vi "AT1B_Ultraschall.vi"() -> ()   [LabVIEW 2026]
doc: "Virtueller Sensor. Teach-Taste einschalten = halten, ausschalten = loslassen. Messgeraeteskala bleibt fest. Bewegung, Messung und Aufnahme sind getrennt schaltbar.\nModellgrenzen stehen in der Anleitung."
panel:
  out "Bewegungsparameter gueltig":bool=TRUE
  out "Grafikfehlercode":i32
  out "Stromverlauf [mA] - 20 ms je Punkt":dbl(graph)
  out "CSV-Fehlercode":i32
  out "Ungespeicherte Daten":bool
  out "Zeilen aufgenommen":i32
  out "Aufnahmestatus":string
  in  "Pruefstand beenden":bool
  in  "Neue CSV-Datei":path
  in  "CSV speichern":bool
  in  "Ungespeicherte Aufnahme verwerfen erlauben":bool
  in  "Neue Aufnahme":bool
  in  "Aufnahme eingeschaltet":bool
  out "Schaltausgang invertiert":bool
  out "Signalzustand":string="Mit Ausfuehren / Strg+R starten."
  out "Messung angehalten - Anzeige historisch":bool
  out "Status-LED":bool
  out "Status-LED [Hz]":dbl=nan
  out "Taste gehalten [s]":dbl=nan
  out "Teach-Phase [0 / 1 / 2]":dbl=nan
  out "Echo-LED":bool
  out "OUT1 - orange":bool
  out "Messgeraet [mm] - feste Skala":dbl=nan
  out "Strom [mA]":dbl=nan
  in  "Messung eingeschaltet":bool=TRUE
  in  "Rausch-Startwert [1..2147483646]":dbl=1.0
  in  "Schalthysterese [mm] - Beispiel":dbl=3.0
  in  "Rauschamplitude [mm] - Beispiel":dbl
  in  "Messoffset [mm] - Beispiel":dbl
  in  "Teach-Taste gedrueckt":bool
  in  "Echo vorhanden":bool=TRUE
  in  "Sensor eingeschaltet":bool=TRUE
  out "Abgeschlossene Fahrten":dbl
  out "Fahrt aktiv":bool
  out "Position aktuell":dbl
  in  "Bewegung pausieren":bool
  in  "Bewegung stoppen":bool
  in  "Ablauf starten":bool
  in  "Schrittweite":dbl=1.0
  in  "Fahrtart":enum16{"Pendeln", "Schritte", "Einfachfahrt"}(ring)
  in  "Wiederholungen":dbl=1.0
  in  "Haltezeit [s]":dbl=0.5
  in  "Tempo pro Sekunde":dbl=25.0
  in  "Endposition":dbl=400.0
  in  "Startposition":dbl=50.0
  in  "Position setzen":bool
  in  "Handposition":dbl=250.0
  out "Kurzhilfe":string="Virtueller Sensor. Teach-Taste einschalten = halten, ausschalten = loslassen. Messgeraeteskala bleibt fest. Bewegung, Messung und Aufnahme sind getrennt schaltbar.\nModellgrenzen stehen in der Anleitung."
  out "Pruefstand":string="AT-1B / Ultraschall AU004 - Wegwerte in mm"
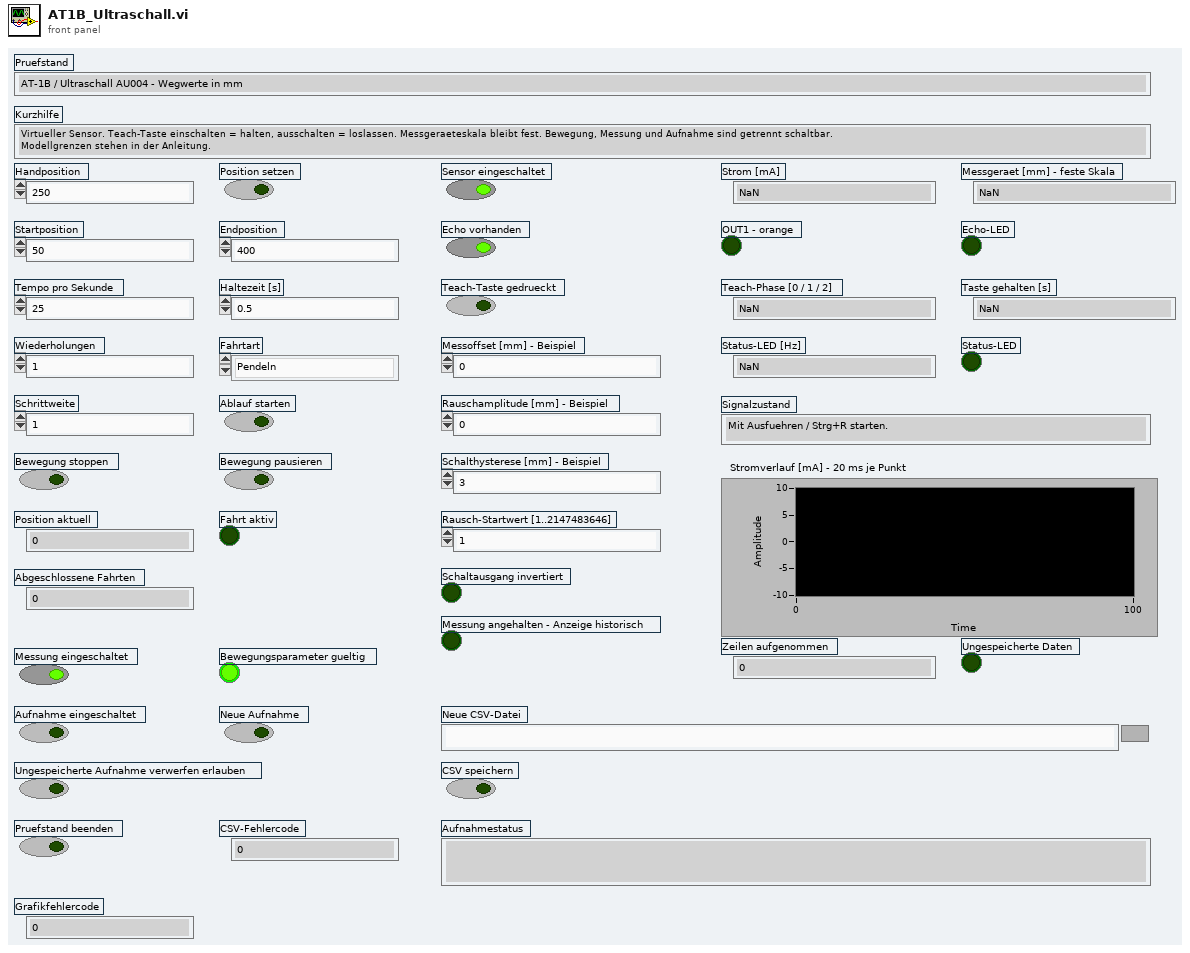
[diagram p1: front panel]
types:
  T1 = cluster{"record":bool, "clear":bool, "limit":i32, "header":string, "source":string}
diagram:
  n1 = while {
    shift-right: [w27] -> _
    shift-left: dbl[] [0.0, 0.0, 0.0, 0.0, 0.0, 0.0, 0.0, 0.0, 0.0, 0.0, 0.0, 0.0] -> [w26]
    shift-right: [w75] -> _
    shift-left: dbl[] [0.0, 0.0, 0.0, 0.0, 0.0, 0.0, 0.0, 0.0, 0.0, 0.0, 0.0, 0.0, 0.0, 0.0, 0.0, 0.0] -> [w74]
    shift-right: [w80] -> _
    shift-left: dbl[] [nan, nan, nan, nan, nan, nan, nan, nan] -> [w79]
    shift-right: [w162] -> _
    shift-left: cluster{"text":string, "count":i32} {"text"="Quelle;Zeit_s;Position_mm;Strom_mA;Anzeige_mm;OUT1;EchoLED;Qualitaet;Teachphase;Taste_s;LED_Hz;Invertiert;StatusLED;Eingang_dt_s;Eingang_distance_mm;Eingang_echo_present;Eingang_power;Eingang_teach_pressed;Eingang_offset_mm;Eingang_noise_amplitude_mm;Eingang_resolution_mm;Eingang_hysteresis_mm_example;Eingang_teach_timeout_s_example;Eingang_noise_seed\r\n", "count"=0} -> [w161]
    shift-right: [w164] -> _
    shift-left: 0 -> [w163]
    shift-right: [w207] -> _
    shift-left: errorcluster {"status"=FALSE, "code"=0, "source"=""} -> [w206]
    i -> [w7]
    stop <- w223 stop-if-true
    w10 = FALSE
    (unwired) 1.0
    w9 = 0.0
    w8 = 0.02
    # "Virtueller Pruefstand - 20 ms Modellschritt"
    n2 = case shown="True" "Position setzen" {
      frame False {
      }
      frame True {
        n3 = property on="Position setzen" class="Bool. (strikt)"("Value"=FALSE) -> ()  [unwired: 2 in, 2 out]
      }
    }
    n4 = case shown="True" "Ablauf starten" {
      frame False {
      }
      frame True {
        n5 = property on="Ablauf starten" class="Bool. (strikt)"("Value"=FALSE) -> ()  [unwired: 2 in, 2 out]
      }
    }
    n6 = case shown="True" "Bewegung stoppen" {
      frame False {
      }
      frame True {
        n7 = property on="Bewegung stoppen" class="Bool. (strikt)"("Value"=FALSE) -> ()  [unwired: 2 in, 2 out]
      }
    }
    n8 = case shown="True" "Neue Aufnahme" {
      frame False {
      }
      frame True {
        n9 = property on="Neue Aufnahme" class="Bool. (strikt)"("Value"=FALSE) -> ()  [unwired: 2 in, 2 out]
      }
    }
    n10 = case shown="True" "CSV speichern" {
      frame False {
      }
      frame True {
        n11 = property on="CSV speichern" class="Bool. (strikt)"("Value"=FALSE) -> ()  [unwired: 2 in, 2 out]
      }
    }
    n12 = case shown="True" "Pruefstand beenden" {
      frame False {
      }
      frame True {
        n13 = property on="Pruefstand beenden" class="Bool. (strikt)"("Value"=FALSE) -> ()  [unwired: 2 in, 2 out]
      }
    }
    n14 = Wait (ms)(milliseconds to wait=u32 20) -> ()  [unwired: 1 out]
    n15 = Select(t=1.0, s="Ablauf starten", f=0.0) -> (s? t:f=w30:dbl)
    n16 = Select(t=1.0, s="Bewegung pausieren", f=0.0) -> (s? t:f=w33:dbl)
    n17 = Select(t=1.0, s="Position setzen", f=0.0) -> (s? t:f=w36:dbl)
    n18 = Select(t=1.0, s="Bewegung stoppen", f=0.0) -> (s? t:f=w39:dbl)
    n19 = Select(t=1.0, s="Echo vorhanden", f=0.0) -> (s? t:f=w65:dbl)
    n20 = property on="Stromverlauf [mA] - 20 ms je Punkt" class="SVDiagr (strikt)"("Legend:Visible"=w10, "Palette:Visible"=w10, "Scale Legend:Visible"=w10, "Position"=cluster{"Left":i32, "Top":i32} {"Left"=735, "Top"=420}, "Plot Area:Size"=cluster{"Width":u32, "Height":u32} {"Width"=340, "Height"=110}) -> (error out=w241:errorcluster)  [unwired: 2 in, 1 out]
    n21 = Select(t=1.0, s="Sensor eingeschaltet", f=0.0) -> (s? t:f=w68:dbl)
    n22 = Select(t=1.0, s="Teach-Taste gedrueckt", f=0.0) -> (s? t:f=w71:dbl)
    n23 = Not(x="Messung eingeschaltet") -> (.not. x?=→"Messung angehalten - Anzeige historisch":bool)
    n24 = And(x="Aufnahme eingeschaltet", y="Messung eingeschaltet") -> (x .and. y?=w173:bool)
    n25 = Unbundle By Name(w161) -> ("count"=w165:i32)  [unwired: 1 out]
    n26 = Equal?(x=w7, y=w9) -> ()  [unwired: 1 out]
    n27 = Quotient & Remainder(x=w7, y=5) -> (x-y*floor(x/y)=w171:i32)  [unwired: 1 out]
    n28 = Build Array(w8, "Startposition", "Endposition", "Tempo pro Sekunde", "Haltezeit [s]", "Wiederholungen", w30, w33, w36, "Handposition", "Fahrtart", "Schrittweite", w39) -> (w40:dbl[])
    n29 = Unbundle By Name(w241) -> ("code"=→"Grafikfehlercode":i32)
    n30 = Greater?(x=w165, y=w163) -> (0:w166:bool)
    n31 = Equal?(x=w171, y=w9) -> (x = y?=w172:bool)
    n32 = call "Trajektorie.vi"("StateIn"=w26, "Parameters"=w40) -> ("Values"=w41:dbl[], "StateOut"=w27:dbl[])  [unwired: 8 in]
    n33 = Not(x=w166) -> (.not. x?=w167:bool)
    n34 = And(x=w173, y=w172) -> (x .and. y?=w174:bool)
    n35 = Index Array(array=w41, index=0) -> (element=w43:dbl)
    "Position aktuell" <- w43
    n36 = Index Array(array=w41, index=3) -> (element=w45:dbl)
    n37 = Index Array(array=w41, index=4) -> (element=w47:dbl)
    n38 = Index Array(array=w41, index=1) -> (element=w51:dbl)
    n39 = Index Array(array=w41, index=2) -> (element=→"Abgeschlossene Fahrten":dbl)
    n40 = Or(x=w167, y="Ungespeicherte Aufnahme verwerfen erlauben") -> (x .or. y?=w168:bool)
    n41 = Greater?(x=w47, y=0.0) -> (0:→"Bewegungsparameter gueltig":bool)
    n42 = Greater?(x=w51, y=0.0) -> (0:→"Fahrt aktiv":bool)
    n43 = Build Array(w8, w43, w65, w68, w71, "Messoffset [mm] - Beispiel", "Rauschamplitude [mm] - Beispiel", 3.0, "Schalthysterese [mm] - Beispiel", 30.0, "Rausch-Startwert [1..2147483646]") -> (w76:dbl[])
    n44 = And(x="Neue Aufnahme", y=w168) -> (x .and. y?=w169:bool)
    n45 = Not(x=w168) -> (.not. x?=w224:bool)
    n46 = call "AU004_Schritt.vi"("StateIn"=w74, "Parameters"=w76) -> ("Values"=w77:dbl[], "StateOut"=w75:dbl[])  [unwired: 8 in]
    n47 = Index Array(array=w76, index=0) -> (element=w181:dbl)
    n48 = Index Array(array=w76, index=1) -> (element=w183:dbl)
    n49 = Index Array(array=w76, index=2) -> (element=w185:dbl)
    n50 = Index Array(array=w76, index=3) -> (element=w187:dbl)
    n51 = Index Array(array=w76, index=4) -> (element=w189:dbl)
    n52 = Index Array(array=w76, index=5) -> (element=w191:dbl)
    n53 = Index Array(array=w76, index=6) -> (element=w193:dbl)
    n54 = Index Array(array=w76, index=7) -> (element=w195:dbl)
    n55 = Index Array(array=w76, index=8) -> (element=w197:dbl)
    n56 = Index Array(array=w76, index=9) -> (element=w199:dbl)
    n57 = Index Array(array=w76, index=10) -> (element=w201:dbl)
    n58 = Bundle By Name(cluster=T1 {"record"=FALSE, "clear"=FALSE, "limit"=10000, "header"="", "source"=""}, "record"=w174, "clear"=w169, "limit"=10000, "header"="Quelle;Zeit_s;Position_mm;Strom_mA;Anzeige_mm;OUT1;EchoLED;Qualitaet;Teachphase;Taste_s;LED_Hz;Invertiert;StatusLED;Eingang_dt_s;Eingang_distance_mm;Eingang_echo_present;Eingang_power;Eingang_teach_pressed;Eingang_offset_mm;Eingang_noise_amplitude_mm;Eingang_resolution_mm;Eingang_hysteresis_mm_example;Eingang_teach_timeout_s_example;Eingang_noise_seed\r\n", "source"="AT1B_Ultraschall;") -> (w179:T1)
    n59 = Select(t=errorcluster {"status"=FALSE, "code"=0, "source"=""}, s=w169, f=w206) -> (s? t:f=w212:errorcluster)
    n60 = Select(t=0, s=w169, f=w163) -> (s? t:f=w219:i32)
    n61 = And(x="Neue Aufnahme", y=w224) -> (x .and. y?=w225:bool)
    n62 = Select(t=w77, s="Messung eingeschaltet", f=w79) -> (s? t:f=w80:dbl[])
    n63 = Index Array(array=w77, index=3) -> (element=w86:dbl)
    n64 = Index Array(array=w77, index=4) -> (element=w90:dbl)
    n65 = Index Array(array=w77, index=14) -> (element=w100:dbl)
    n66 = Index Array(array=w77, index=5) -> (element=w105:dbl)
    n67 = Index Array(array=w77, index=12) -> (element=w132:dbl)
    n68 = Index Array(array=w77, index=0) -> (element=w136:dbl)
    n69 = Index Array(array=w77, index=1) -> (element=w138:dbl)
    n70 = Index Array(array=w77, index=3) -> (element=w140:dbl)
    n71 = Index Array(array=w77, index=4) -> (element=w142:dbl)
    n72 = Index Array(array=w77, index=5) -> (element=w144:dbl)
    n73 = Index Array(array=w77, index=6) -> (element=w146:dbl)
    n74 = Index Array(array=w77, index=7) -> (element=w148:dbl)
    n75 = Index Array(array=w77, index=8) -> (element=w150:dbl)
    n76 = Index Array(array=w77, index=12) -> (element=w152:dbl)
    n77 = Index Array(array=w77, index=14) -> (element=w154:dbl)
    n78 = Index Array(array=w80, index=0) -> (element=→"Strom [mA]":dbl)
    n79 = Index Array(array=w80, index=1) -> (element=→"Messgeraet [mm] - feste Skala":dbl)
    n80 = Greater?(x=w86, y=0.0) -> (0:→"OUT1 - orange":bool)
    n81 = Greater?(x=w90, y=0.0) -> (0:→"Echo-LED":bool)
    n82 = Index Array(array=w80, index=6) -> (element=→"Teach-Phase [0 / 1 / 2]":dbl)
    n83 = Index Array(array=w80, index=7) -> (element=→"Taste gehalten [s]":dbl)
    n84 = Index Array(array=w80, index=8) -> (element=→"Status-LED [Hz]":dbl)
    n85 = Greater?(x=w100, y=0.0) -> (0:→"Status-LED":bool)
    n86 = Equal?(x=w105, y=0.0) -> (x = y?=w108:bool)
    n87 = Equal?(x=w105, y=1.0) -> (x = y?=w112:bool)
    n88 = Equal?(x=w105, y=2.0) -> (x = y?=w116:bool)
    n89 = Equal?(x=w105, y=3.0) -> (x = y?=w120:bool)
    n90 = Equal?(x=w105, y=4.0) -> (x = y?=w124:bool)
    n91 = Equal?(x=w105, y=5.0) -> (x = y?=w128:bool)
    n92 = Greater?(x=w132, y=0.0) -> (0:→"Schaltausgang invertiert":bool)
    n93 = Build Array(w45, w43, w136, w138, w140, w142, w144, w146, w148, w150, w152, w154, w181, w183, w185, w187, w189, w191, w193, w195, w197, w199, w201) -> (w202:dbl[])
    n94 = Index Array(array=w80, index=0) -> (element=→"Stromverlauf [mA] - 20 ms je Punkt":dbl)
    n95 = Select(t="Messsignal gueltig", s=w108, f="Parameter ungueltig - Eingaben pruefen.") -> (s? t:f=w110:string)
    n96 = call "Aufzeichnung_Schritt.vi"("Previous"=w161, "Row"=w202, "Settings"=w179) -> ("Full"=w203:bool, "Current"=w162:cluster{"text":string, "count":i32})  [unwired: 11 in]
    n97 = Select(t="Noch keine Teachpunkte gespeichert", s=w112, f=w110) -> (s? t:f=w114:string)
    n98 = Unbundle By Name(w162) -> ("text"=w204:string, "count"=w205:i32)
    "Zeilen aufgenommen" <- w205
    n99 = Select(t="Abstand ausserhalb 50..400 mm", s=w116, f=w114) -> (s? t:f=w118:string)
    n100 = Greater?(x=w205, y=0.0) -> (0:w209:bool)
    n101 = Select(t="Kein Echo", s=w120, f=w118) -> (s? t:f=w122:string)
    n102 = And(x="CSV speichern", y=w209) -> (x .and. y?=w210:bool)
    n103 = case shown="True" w210 {
      tunnel: "Neue CSV-Datei" -> [_ w244]
      tunnel: w212 -> [w243 _]
      tunnel: w204 -> [_ w245]
      tunnel: [w243 w246] -> w207
      frame False {
      }
      frame True {
        n104 = call "CSV_Speichern.vi"("Text"=w245, "Datei"=w244) -> ("error out"=w246:errorcluster)  [unwired: 13 in]
      }
    }
    n105 = Select(t="Sensor laeuft an", s=w124, f=w122) -> (s? t:f=w126:string)
    n106 = Select(t="Sensor ausgeschaltet", s=w128, f=w126) -> (s? t:f=→"Signalzustand":string)
    n107 = Unbundle By Name(w207) -> ("status"=w213:bool, "code"=→"CSV-Fehlercode":i32, "source"=w215:string)
    n108 = Not(x=w213) -> (.not. x?=w216:bool)
    n109 = And(x=w210, y=w216) -> (x .and. y?=w217:bool)
    n110 = Select(t=w205, s=w217, f=w219) -> (s? t:f=w164:i32)
    n111 = Greater?(x=w205, y=w164) -> (0:w220:bool)
    "Ungespeicherte Daten" <- w220
    n112 = Not(x=w220) -> (.not. x?=w221:bool)
    n113 = Select(t="Aufnahme noch nicht gespeichert. Vor neuer Aufnahme oder Beenden CSV speichern oder Verwerfen erlauben einschalten.", s=w220, f="Bereit. Aufnahme mit neuem Dateinamen speichern.") -> (s? t:f=w231:string)
    n114 = Or(x=w221, y="Ungespeicherte Aufnahme verwerfen erlauben") -> (x .or. y?=w222:bool)
    n115 = Select(t="Aufnahme voll (10 000 Zeilen). Speichern und neue Aufnahme beginnen.", s=w203, f=w231) -> (s? t:f=w233:string)
    n116 = And(x="Pruefstand beenden", y=w222) -> (x .and. y?=w223:bool)
    n117 = Not(x=w223) -> (.not. x?=w226:bool)
    n118 = And(x="Pruefstand beenden", y=w226) -> (x .and. y?=w227:bool)
    n119 = Or(x=w225, y=w227) -> (x .or. y?=w228:bool)
    n120 = Select(t="Erst CSV speichern oder Verwerfen erlauben einschalten.", s=w228, f=w233) -> (s? t:f=w235:string)
    n121 = Select(t=w215, s=w213, f=w235) -> (s? t:f=→"Aufnahmestatus":string)
    "Pruefstand" <- "AT-1B / Ultraschall AU004 - Wegwerte in mm"
    "Kurzhilfe" <- "Virtueller Sensor. Teach-Taste einschalten = halten, ausschalten = loslassen. Messgeraeteskala bleibt fest. Bewegung, Messung und Aufnahme sind getrennt schaltbar.\nModellgrenzen stehen in der Anleitung."
  }
